vi "handle_requests.vi"(8 "error in":errorcluster, 9 "Python env version":string="3.12", 10 "Path to service.py":path, 11 "Python env directory":path) -> (0 "error out":errorcluster)   [LabVIEW 2023]
uses:
  <vilib>/Python/Open Venv Python Session.vi
panel:
  in  "Process Stop Button":bool
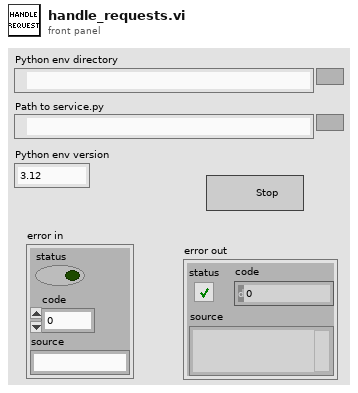
[diagram p1: front panel]
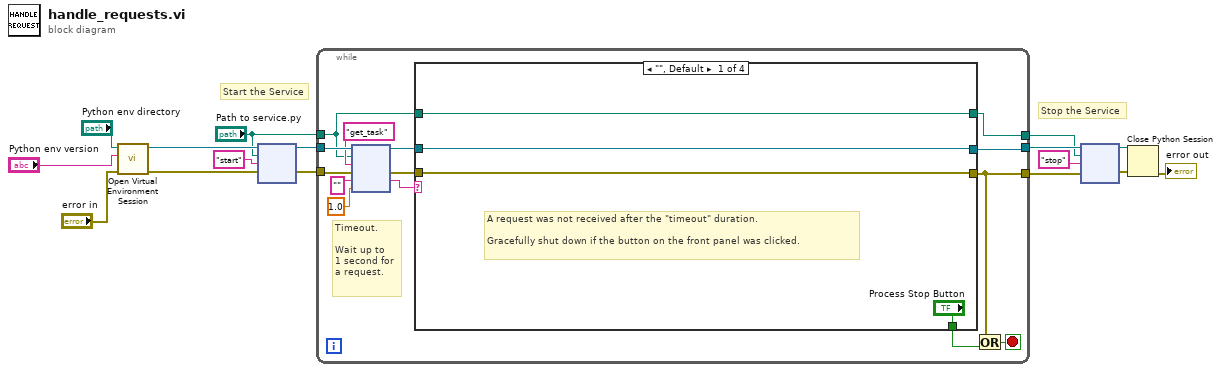
[diagram p0: block diagram]
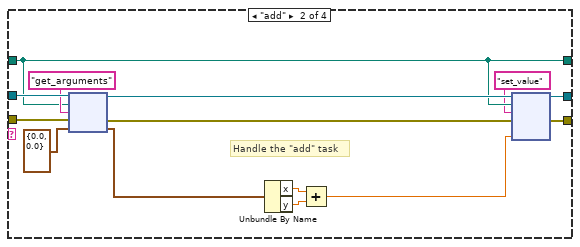
[diagram p2: hidden frame]
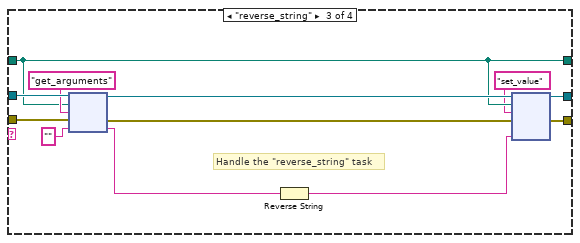
[diagram p3: hidden frame]
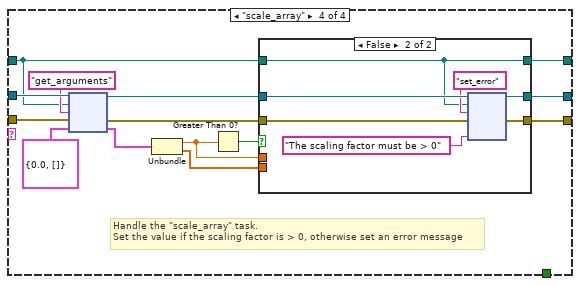
[diagram p4: hidden frame]
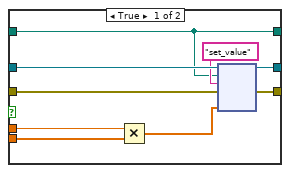
[diagram p5: hidden frame]
diagram:
  # "Stop the Service"
  # "Start the Service"
  n1 = call-poly <vilib>:"Open Virtual Environment Session.vi"("error in (no error)"="error in", "Python version"="Python env version", "Env path"="Python env directory") -> ("error out"=w13:errorcluster, "session out"=w14:refnum<k35>)  [unwired: 7 in]
  n2 = node(w14, "Path to service.py", "start" ("function name"), w13) -> (w10:refnum<k35>, w11:errorcluster)  [unwired: 2 in, 2 out]
  n3 = while {
    tunnel: w11 -> [w29]
    tunnel: w10 -> [w28]
    tunnel: [w18] -> w9
    tunnel: [w19] -> w8
    tunnel: "Path to service.py" -> [w20]
    tunnel: [w17] -> w5
    stop <- w30 stop-if-true
    # "Timeout.\n\nWait up to \n1 second for\na request."
    n4 = node(w28, w20, "get_task" ("function name"), w29, "" ("return type"), 1.0) -> (w21:refnum<k35>, w23:errorcluster, w25:string)  [unwired: 1 in, 2 out]
    n5 = case shown="\"\", Default" w25 {
      tunnel: w23 -> [w33 w46 w58 w72]
      tunnel: ["Process Stop Button" _ _ _] -> w22
      tunnel: w21 -> [w32 w48 w60 w74]
      tunnel: w20 -> [w31 w37 w53 w67]
      tunnel: [w33 w39 w55 w69] -> w19
      tunnel: [w32 w38 w54 w68] -> w18
      tunnel: [w31 w37 w53 w61] -> w17
      frame "", Default {
        # "A request was not received after the \"timeout\" duration.\n\nGracefully shut down if the button on the front panel was clicked."
      }
      frame "add" {
        # "Handle the \"add\" task"
        n6 = node(w48, w37, "get_arguments" ("function name"), w46, cluster{"x":dbl, "y":dbl} {"x"=0.0, "y"=0.0}) -> (w41:refnum<k35>, w40:errorcluster, w44:cluster{"x":dbl, "y":dbl})  [unwired: 2 out]
        n7 = Unbundle By Name(w44) -> ("x"=w43:dbl, "y"=w42:dbl)
        n8 = Add(x=w43, y=w42) -> (x+y=w36:dbl)
        n9 = node(w41, w37, "set_value" ("function name"), w40, w36) -> (w38:refnum<k35>, w39:errorcluster)  [unwired: 3 in, 2 out]
      }
      frame "reverse_string" {
        # "Handle the \"reverse_string\" task"
        n10 = node(w60, w53, "get_arguments" ("function name"), w58, "" ("return type")) -> (w57:refnum<k35>, w56:errorcluster, w50:string)  [unwired: 2 out]
        n11 = Reverse String(1:w50) -> (0:w49:string)
        n12 = node(w57, w53, "set_value" ("function name"), w56, w49) -> (w54:refnum<k35>, w55:errorcluster)  [unwired: 3 in, 2 out]
      }
      frame "scale_array" {
        # "Handle the \"scale_array\" task.\nSet the value if the scaling factor is > 0, otherwise set an error message"
        n13 = node(w74, w67, "get_arguments" ("function name"), w72, cluster{dbl, dbl[]} {0.0, []}) -> (w71:refnum<k35>, w70:errorcluster, w65:cluster{dbl, dbl[]})  [unwired: 2 out]
        n14 = Unbundle(w65) -> (w62:dbl, w63:dbl[])
        n15 = Greater Than 0?(x=w62) -> (x > 0?=w64:bool)
        n16 = case shown="False" w64 {
          tunnel: w71 -> [w83 w90]
          tunnel: w70 -> [w82 w89]
          tunnel: [w81 w88] -> w69
          tunnel: [w80 w87] -> w68
          tunnel: w67 -> [w75 w84]
          tunnel: w63 -> [w78 _]
          tunnel: w62 -> [w77 _]
          tunnel: [w75 w84] -> w61
          frame True {
            n17 = Multiply(x=w77, y=w78) -> (x*y=w76:dbl[])
            n18 = node(w83, w75, "set_value" ("function name"), w82, w76) -> (w80:refnum<k35>, w81:errorcluster)  [unwired: 3 in, 2 out]
          }
          frame False {
            n19 = node(w90, w84, "set_error" ("function name"), w89, "The scaling factor must be > 0") -> (w87:refnum<k35>, w88:errorcluster)  [unwired: 3 in, 2 out]
          }
        }
      }
    }
    n20 = Or(x=w19, y=w22) -> (x .or. y?=w30:bool)
  }
  n21 = node(w9, w5, "stop" ("function name"), w8) -> (w4:refnum<k35>, w1:errorcluster)  [unwired: 2 in, 2 out]
  n22 = Close Python Session(session in=w4, error in=w1) -> (11:→"error out":errorcluster)
